vi "Get all IDs.vi"(8 "error in (no error)":errorcluster, 11 "Guardian List in":refnum<class "Guardian List.lvclass">) -> (0 "error out":errorcluster, 2 "All IDs":string[](array[string]), 3 "Guardian List out":refnum<class "Guardian List.lvclass">)   [LabVIEW 2020, in "TALOS.lvlib" / "Classes.lvlib" / "Guardian List.lvclass"]
uses:
  Guardian List.lvclass
  Guardian List.lvclass/Guardian List.ctl
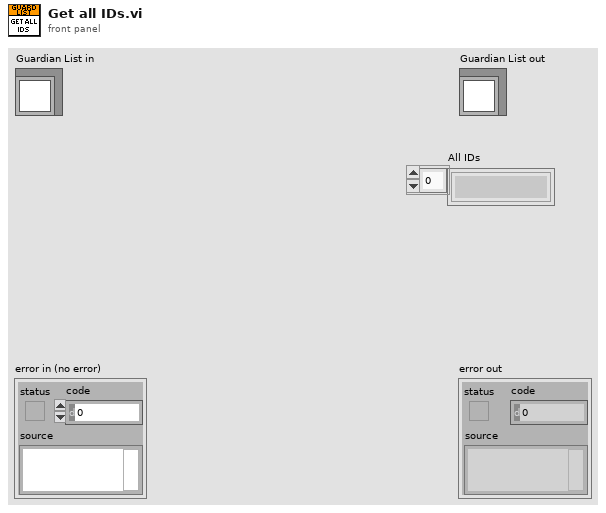
[diagram p1: front panel]
types:
  T1 = typedef "TALOS.lvlib/Classes.lvlib/Guardian List.lvclass/Guardian Properties.ctl" = cluster{"Alive":bool, "Last Seen":timestamp, "Guardian Health":refnum<class "AEgIS Shared Variables.lvclass">, "Guardian Message":refnum<class "AEgIS Shared Variables.lvclass">, "IP":string, "TCP Writer associated ID":string, "uS List received":bool}
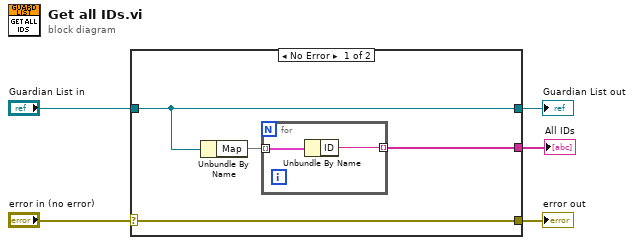
[diagram p0: block diagram]
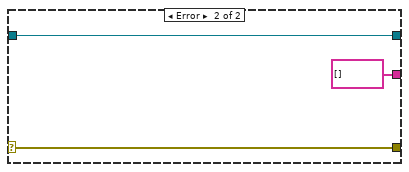
[diagram p2: hidden frame]
diagram:
  n1 = case shown="No Error" "error in (no error)" {
    selector: "error in (no error)" -> [w9 w14]
    tunnel: [w9 w14] -> w4
    tunnel: [w8 w13] -> w2
    tunnel: "Guardian List in" -> [w8 w13]
    tunnel: [w6 string[] []] -> w1
    frame No Error {
      n2 = Unbundle By Name(w8) -> ("Map"=w7:map{string, T1})
      n3 = for {
        tunnel: w7 -> [w11] mode=indexing
        tunnel: [w10] -> w6 mode=indexing
        n4 = Unbundle By Name(w11) -> ("ID"=w10:string)
      }
    }
    frame Error {
    }
  }
  "error out" <- w4
  "Guardian List out" <- w2
  "All IDs" <- w1
